vi "load_test_plan.vi"(6 "error in load_test":errorcluster, 8 "Power W":dbl, 9 "Speed RPM":dbl, 10 "Session":dbl, 11 "Plan File":path) -> (0 "Reference":i32[](array[numeric]), 1 "Resistor":i32[](array[numeric]), 2 "Arms":i32[](array[numeric]), 3 "N Tests":i32, 4 "error out load_test":errorcluster)   [LabVIEW 2025]
uses:
  <vilib>/Utility/file.llb/Read Delimited Spreadsheet (string).vi
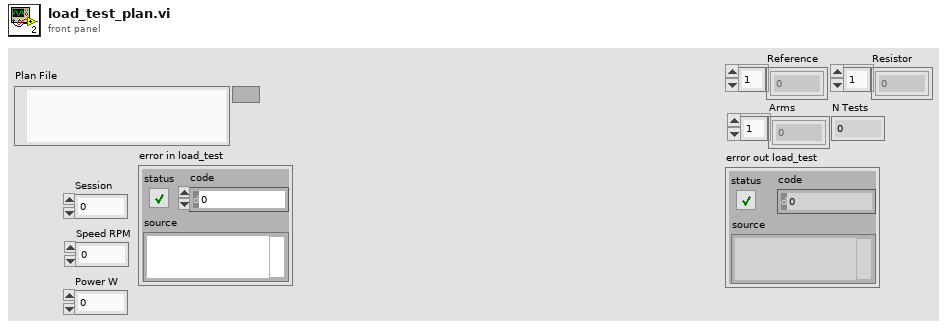
[diagram p1: front panel]
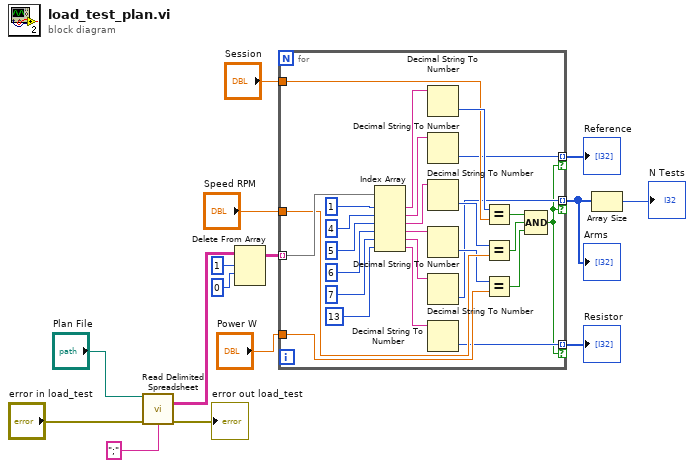
[diagram p0: block diagram]
diagram:
  n1 = call-poly <vilib>:"Read Delimited Spreadsheet.vi"("file path (dialog if empty)"="Plan File", "error in (no error)"="error in load_test", "delimiter (\\t)"=";" ("delimiter (\\t)")) -> ("all rows"=w13:string[][], "error out"=→"error out load_test":errorcluster)  [unwired: 7 in, 4 out]
  n2 = Delete From Array(array=w13, length=1, index (row)=0) -> (array with subset deleted=w10:string[][])  [unwired: 1 in, 1 out]
  n3 = for {
    tunnel: w10 -> [w35] mode=indexing
    tunnel: "Session" -> [w27]
    tunnel: "Power W" -> [w23]
    tunnel: "Speed RPM" -> [w25]
    tunnel: [w22] -> w6 mode=indexing if=w16
    tunnel: [w21] -> w4 mode=indexing if=w16
    tunnel: [w20] -> w5 mode=indexing if=w16
    n4 = Index Array(array=w35, index #1=1 ("index"), index #2=4 ("index"), index #3=5 ("index"), index #4=6 ("index"), index #5=7 ("index"), index #6=13 ("index")) -> (element #1=w34:string, element #2=w33:string, element #3=w32:string, element #4=w31:string, element #5=w30:string, element #6=w29:string)
    n5 = Decimal String To Number(string=w34) -> (number=w28:i32)  [unwired: 2 in, 1 out]
    n6 = Decimal String To Number(string=w33) -> (number=w22:i32)  [unwired: 2 in, 1 out]
    n7 = Decimal String To Number(string=w32) -> (number=w26:i32)  [unwired: 2 in, 1 out]
    n8 = Decimal String To Number(string=w31) -> (number=w24:i32)  [unwired: 2 in, 1 out]
    n9 = Decimal String To Number(string=w30) -> (number=w21:i32)  [unwired: 2 in, 1 out]
    n10 = Decimal String To Number(string=w29) -> (number=w20:i32)  [unwired: 2 in, 1 out]
    n11 = Equal?(x=w28, y=w27) -> (x = y?=w19:bool)
    n12 = Equal?(x=w26, y=w25) -> (x = y?=w18:bool)
    n13 = Equal?(x=w24, y=w23) -> (x = y?=w17:bool)
    n14 = Compound Arithmetic op=AND(w19, w18, w17) -> (w16:bool)
  }
  "Reference" <- w6
  "Arms" <- w4
  "Resistor" <- w5
  n15 = Array Size(array=w4) -> (size(s)=→"N Tests":i32)
